vi "DAC Configure.vi"(8 "error in":errorcluster, 11 "DAC Keller BNC in":refnum<class "DAC Keller BNC.lvclass">) -> (0 "error out":errorcluster, 3 "DAC Keller BNC out":refnum<class "DAC Keller BNC.lvclass">)   [LabVIEW 2019, in "DAC.lvlib" / "DAC Keller BNC.lvclass"]
uses:
  DAC Keller BNC.lvclass
  C:/Users/wg/Documents/LV_Projects/test-stand/App/DAC/DAC.lvclass
  DAC.lvclass/DAC.ctl
  DAC Keller BNC.lvclass/DAC Keller BNC.ctl
  <vilib>/DAQmx/create/scale.llb/DAQmx Create Scale (Map Ranges).vi
  <vilib>/DAQmx/create/channels.llb/DAQmx Create Channel (AI-Voltage-Basic).vi
  <vilib>/DAQmx/configure/timing.llb/DAQmx Timing (Sample Clock).vi
  DAC.lvclass
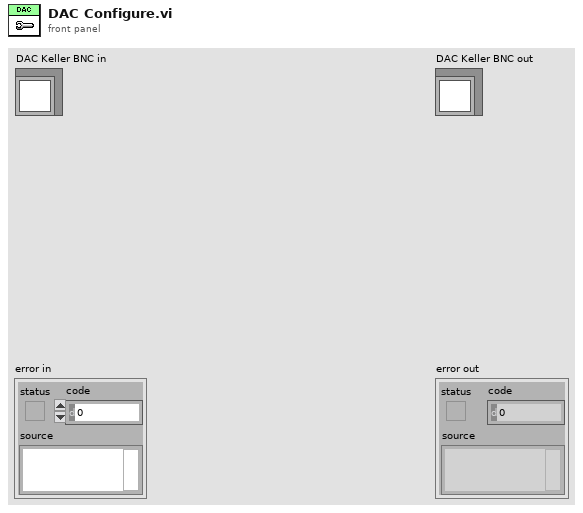
[diagram p1: front panel]
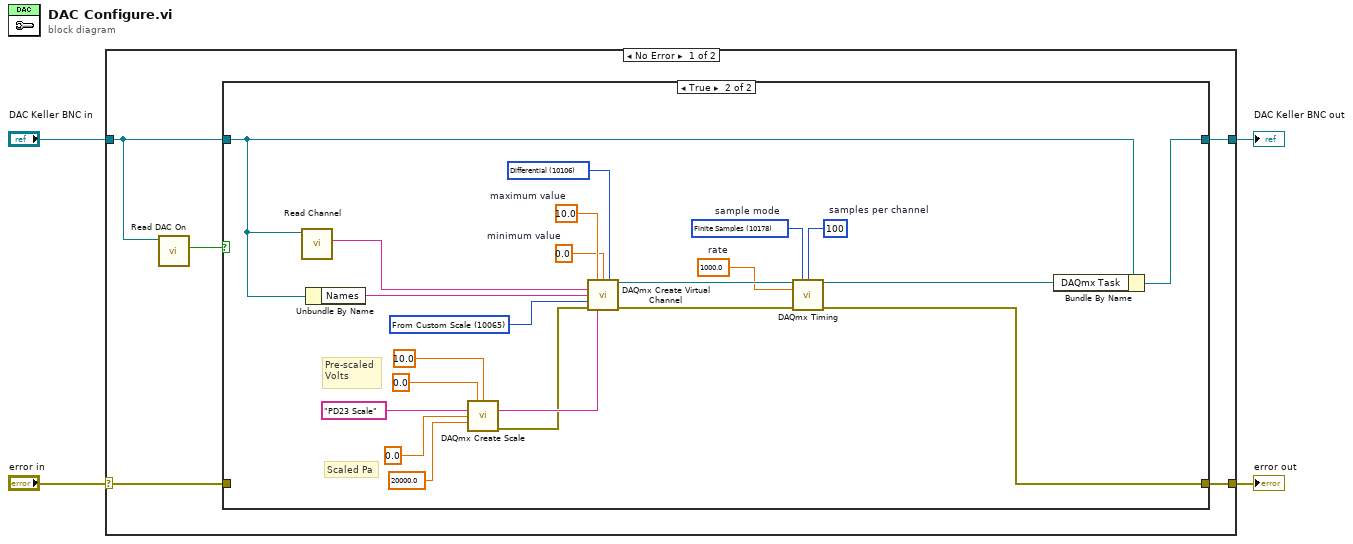
[diagram p0: block diagram]
diagram:
  n1 = case shown="No Error" "error in" {
    selector: "error in" -> [w6 w35]
    tunnel: [w5 w35] -> w4
    tunnel: [w7 w34] -> w3
    tunnel: "DAC Keller BNC in" -> [w9 w34]
    frame No Error {
      n2 = call "Read DAC On.vi"("DAC in"=w9) -> ("DAC On"=w8:bool)  [unwired: 8 in, 2 out]
      n3 = case shown="True" w8 {
        tunnel: w9 -> [w11 w31]
        tunnel: [w11 w33] -> w7
        tunnel: w6 -> [w10 _]
        tunnel: [w10 w12] -> w5
        frame False {
        }
        frame True {
          w21 = 10106 items=["Default"=-1, "RSE"=10083, "NRSE"=10078, "Differential"=10106, "Pseudodifferential"=12529] ("input terminal configuration")
          w22 = 0.0  # minimum value
          w23 = 10.0  # maximum value
          w24 = 100  # samples per channel
          w25 = 1000.0  # rate
          w26 = 10178 items=["Finite Samples"=10178, "Continuous Samples"=10123, "Hardware Timed Single Point"=12522]  # sample mode
          w29 = 10065 items=["Volts"=10348, "From Custom Scale"=10065] ("units")
          # "Scaled Pa"
          # "Pre-scaled\nVolts"
          n4 = call "Read Channel.vi"("DAC in"=w31) -> ("Channel"=w30:string)  [unwired: 8 in, 2 out]
          n5 = Unbundle By Name(w31) -> ("Names"=w32:string)
          n6 = call-poly <vilib>:"DAQmx Create Scale.vi"("pre-scaled minimum"=0.0, "pre-scaled maximum"=10.0, "name"="PD23 Scale", "scaled minimum"=0.0, "scaled maximum"=20000.0) -> ("scale out"=w15:tag, "error out"=w14:errorcluster)  [unwired: 9 in]
          n7 = call-poly <vilib>:"DAQmx Create Virtual Channel.vi"("maximum value"=w23, "minimum value"=w22, "input terminal configuration"=w21, "physical channels"=w30, "name to assign"=w32, "units"=w29, "error in"=w14, "custom scale name"=w15) -> ("task out"=w28:refnum<k21>, "error out"=w27:errorcluster)  [unwired: 6 in]
          n8 = call-poly <vilib>:"DAQmx Timing.vi"("task/channels in"=w28, "sample mode"=w26, "samples per channel"=w24, "rate"=w25, "error in"=w27) -> ("task out"=w13:refnum<k21>, "error out"=w12:errorcluster)  [unwired: 9 in]
          n9 = Bundle By Name(cluster=w31, "DAQmx Task"=w13) -> (w33:refnum<class "DAC Keller BNC.lvclass">)
        }
      }
    }
    frame Error {
    }
  }
  "error out" <- w4
  "DAC Keller BNC out" <- w3
